vi "Get_Input.vi"(8 "error in (no error)":errorcluster, 11 "object in":refnum<class "DIO_Channel.lvclass">) -> (0 "error out":errorcluster, 2 "Input":bool, 3 "object out":refnum<class "DIO_Channel.lvclass">)   [LabVIEW 2021, in "Simulator-Channel.lvlib" / "DIO_Channel.lvclass"]
doc: "Gets the Input"
uses:
  DIO_Channel.lvclass
  C:/Users/averna/Documents/LV Gym DEMO/Factory Pattern/Device Channels/Dependencies/DIO-Channel.lvlibp/Channels/DIO-Channel/DIO_Channel_class/DIO_Channel.lvclass
  DIO_Channel.lvclass/DIO_Channel.ctl
  Panel/DIO_Panel Messages/Get Input Msg/Get Input Msg.lvclass/Get Input Msg.ctl
  <vilib>/ActorFramework/Message Enqueuer/Message Enqueuer.lvclass/Message Enqueuer.ctl
  <vilib>/ActorFramework/Message Enqueuer/Enqueue.vi
  Panel/DIO_Panel Messages/Get Input Msg/Get Input Msg.lvclass
  C:/Program Files/National Instruments/LabVIEW 2021/vi.lib/ActorFramework/Message/Message.lvclass
  Dependencies/DIO-Channel.lvlibp/Channels/DIO-Channel/DIO_Channel_class/Properties/GetDIOConfiguration.vi
  <vilib>/ActorFramework/Message Priority Queue/Priority Enqueue.vi
  Dependencies/DIO-Channel.lvlibp/Channels/DIO-Channel/DIO-Configuration_class/DIO-Configuration.lvclass
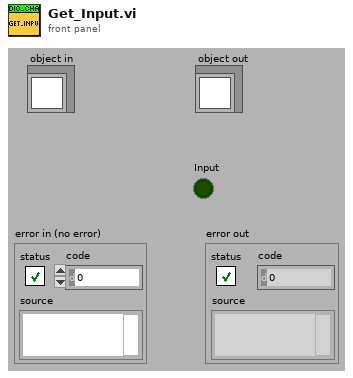
[diagram p1: front panel]
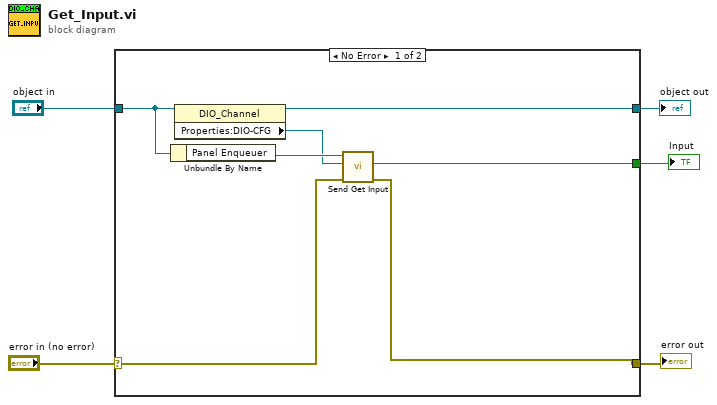
[diagram p0: block diagram]
diagram:
  n1 = case shown="No Error" "error in (no error)" {
    selector: "error in (no error)" -> [w7 w14]
    tunnel: [w6 w14] -> w4
    tunnel: [w10 w13] -> w2
    tunnel: "object in" -> [w12 w13]
    tunnel: [w8 _] -> w1
    frame No Error {
      n2 = Unbundle By Name(w12) -> ("Panel Enqueuer"=w11:refnum<class "Message Enqueuer.lvclass">)
      n3 = property class="DIO_Channel"(reference=w12) -> (reference out=w10:refnum<class "DIO_Channel.lvclass">, "Properties:DIO-CFG"=w9:refnum<class "DIO-Configuration.lvclass">)  [unwired: 1 in, 1 out]
      n4 = call "Send Get Input.vi"("error in (no error)"=w7, "DIO_CFG"=w9, "Message Enqueuer"=w11) -> ("error out"=w6:errorcluster, "Input"=w8:bool)  [unwired: 6 in, 1 out]
    }
    frame Error {
    }
  }
  "error out" <- w4
  "object out" <- w2
  "Input" <- w1
